vi "VIH Project - Get Effective Group Rule - Inherit.vi"(7 "Ignore Control Rules (F)":bool, 10 "Group Rule":T1, 11 "Parent Group Rule":T1) -> (2 "Effective Group Rule":T1)   [LabVIEW 2014]
doc: "::: VI Helpeks :::\nCopyright (c) 2000-2026 Konstantin Shifershteyn. All rights reserved."
uses:
  _VIH HelpGen.llb/VIH HelpGen Typedef - Cluster - Group Rule.ctl
  _VIH HelpGen.llb/VIH HelpGen Typedef - Enum - Default,Enable,Disable.ctl
  _VIH HelpGen.llb/VIH HelpGen Typedef - Cluster - Group Rule - Source Paths.ctl
  _VIH HelpGen.llb/VIH HelpGen Typedef - Cluster - Group Rule - Target Paths.ctl
  _VIH HelpGen.llb/VIH HelpGen Typedef - Enum - Description Mode.ctl
  _VIH HelpGen.llb/VIH HelpGen Typedef - Cluster - Control Rule.ctl
  _VIH HelpGen.llb/VIH HelpGen Typedef - Cluster - Enum Value Info.ctl
  _VIH HelpGen.llb/VIH HelpGen Typedef - Cluster - Group Rule - Flags.ctl
panel:
  # "VI Helpeks\nCopyright (c) 2012-2026 Konstantin Shifershteyn"
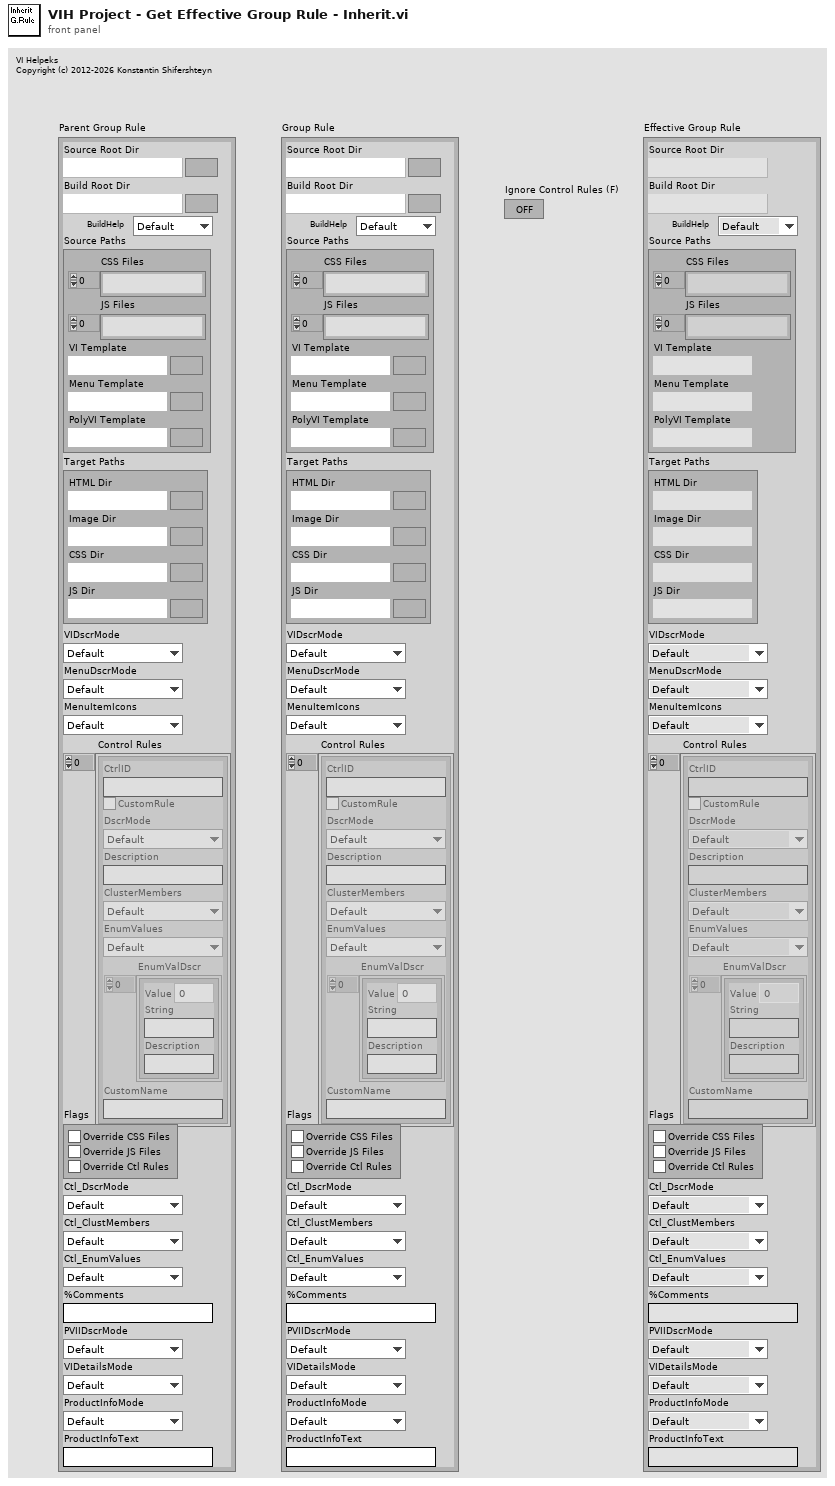
[diagram p1: front panel]
types:
  T1 = typedef "VIH HelpGen Typedef - Cluster - Group Rule.ctl" = cluster{"Source Root Dir":path, "Build Root Dir":path, "BuildHelp":T2, "Source Paths":T3, "Target Paths":T4, "VIDscrMode":T5, "MenuDscrMode":T5, "MenuItemIcons":T2, "Control Rules":T6[], "Flags":T8, "Ctl_DscrMode":T5, "Ctl_ClustMembers":T2, "Ctl_EnumValues":T2, "%Comments":string, "PVIIDscrMode":T5, "VIDetailsMode":T5, "ProductInfoMode":T2, "ProductInfoText":string}
  T2 = typedef "VIH HelpGen Typedef - Enum - Default,Enable,Disable.ctl" = enum16{"Default", "Enable", "Disable"}
  T3 = typedef "VIH HelpGen Typedef - Cluster - Group Rule - Source Paths.ctl" = cluster{"CSS Files":path[], "JS Files":path[], "VI Template":path, "Menu Template":path, "PolyVI Template":path}
  T4 = typedef "VIH HelpGen Typedef - Cluster - Group Rule - Target Paths.ctl" = cluster{"HTML Dir":path, "Image Dir":path, "CSS Dir":path, "JS Dir":path}
  T5 = typedef "VIH HelpGen Typedef - Enum - Description Mode.ctl" = enum16{"Default", "Description", "Description1", "Description2", "Custom", "None"}
  T6 = typedef "VIH HelpGen Typedef - Cluster - Control Rule.ctl" = cluster{"CtrlID":string, "CustomRule":bool, "DscrMode":T5, "Description":string, "ClusterMembers":T2, "EnumValues":T2, "EnumValDscr":T7[], "CustomName":string}
  T7 = typedef "VIH HelpGen Typedef - Cluster - Enum Value Info.ctl" = cluster{"Value":ext, "String":string, "Description":string}
  T8 = typedef "VIH HelpGen Typedef - Cluster - Group Rule - Flags.ctl" = cluster{"Override CSS Files":bool, "Override JS Files":bool, "Override Ctl Rules":bool}
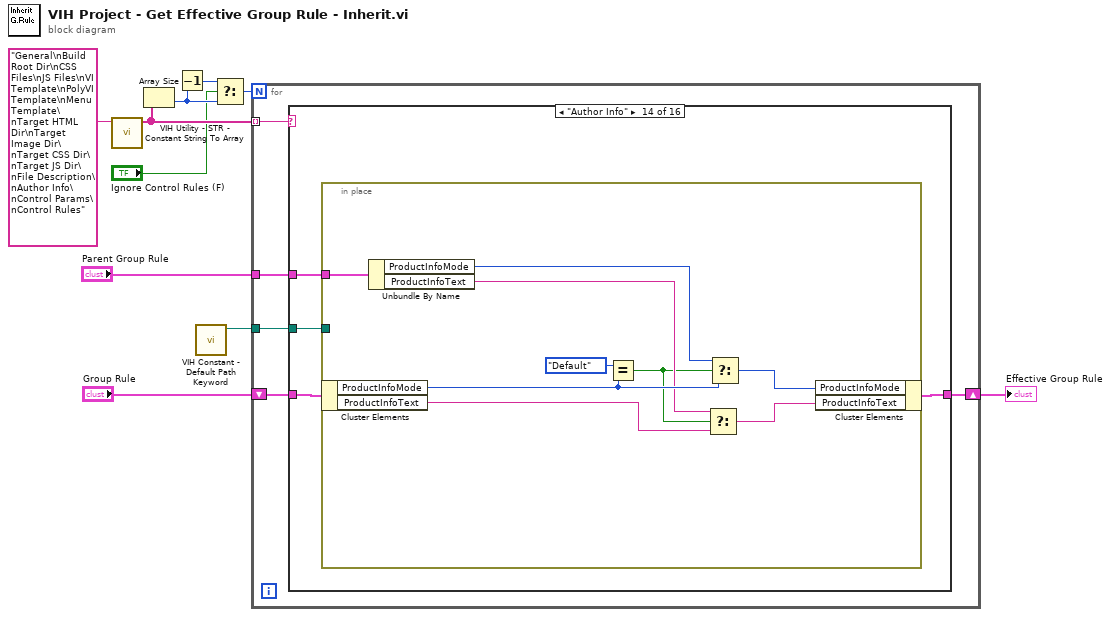
[diagram p0: block diagram]
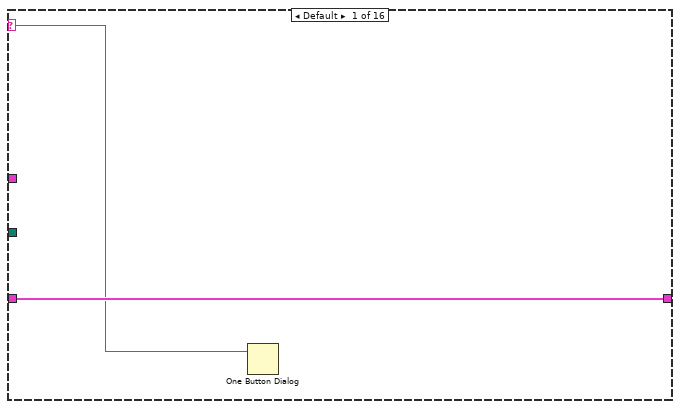
[diagram p2: hidden frame]
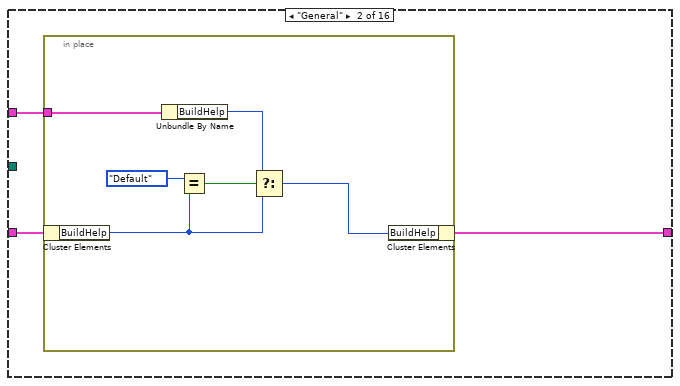
[diagram p3: hidden frame]
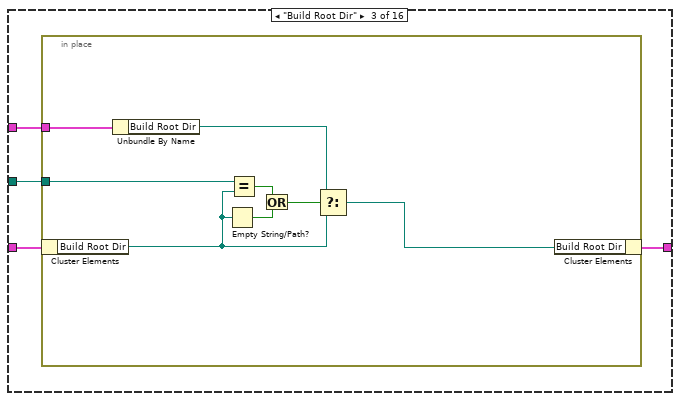
[diagram p4: hidden frame]
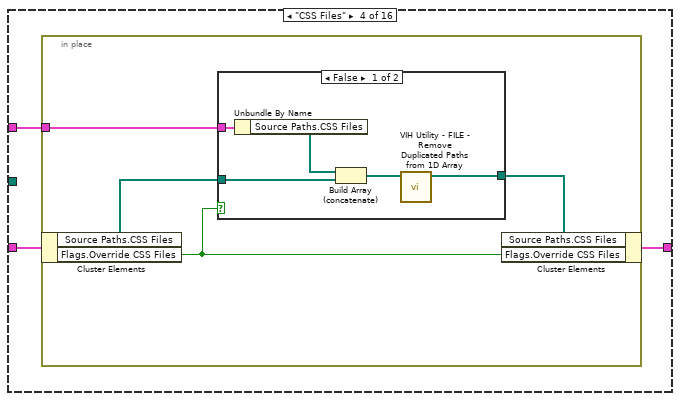
[diagram p5: hidden frame]
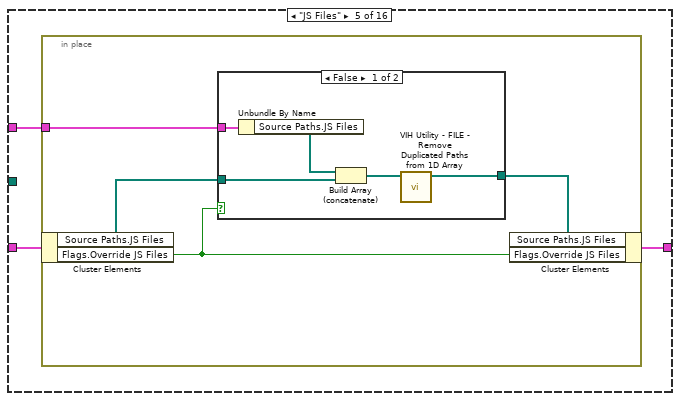
[diagram p7: hidden frame]
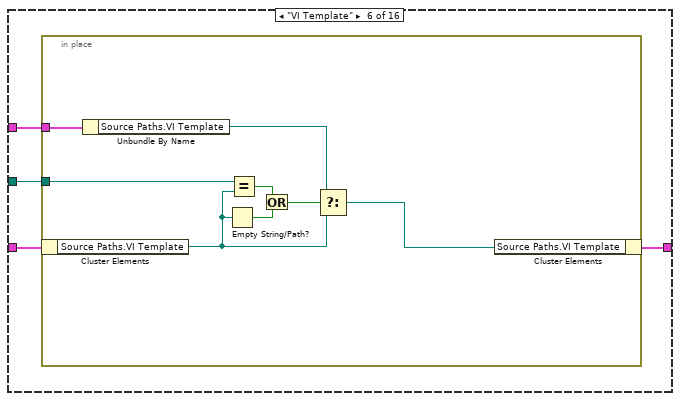
[diagram p9: hidden frame]
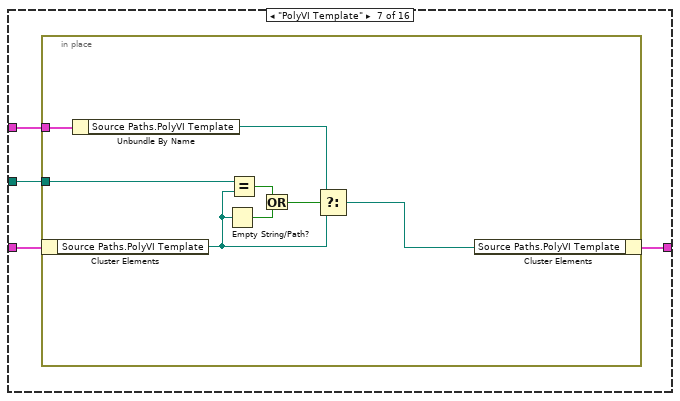
[diagram p10: hidden frame]
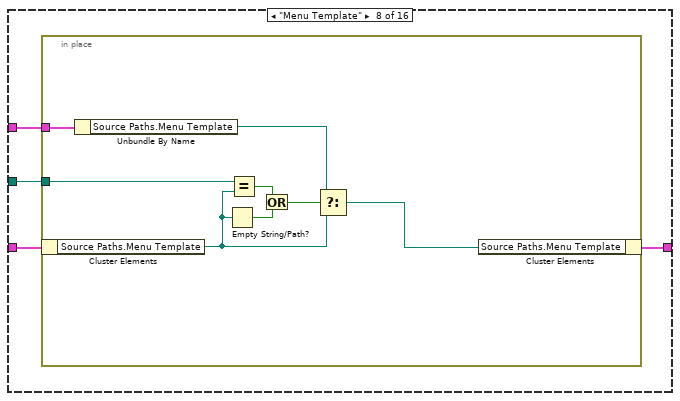
[diagram p11: hidden frame]
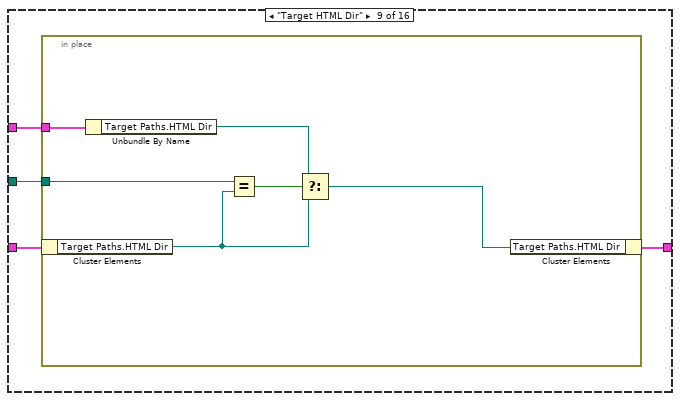
[diagram p12: hidden frame]
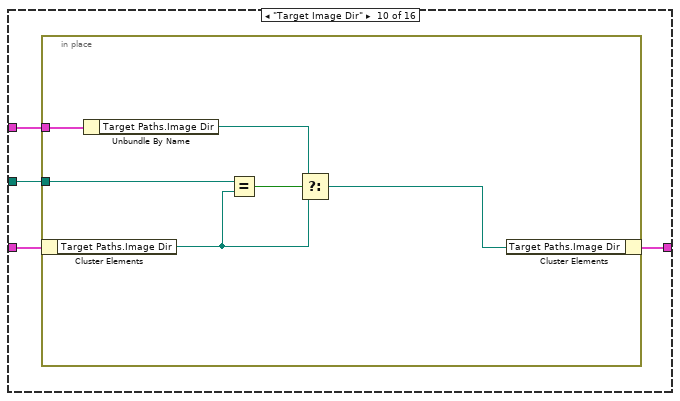
[diagram p13: hidden frame]
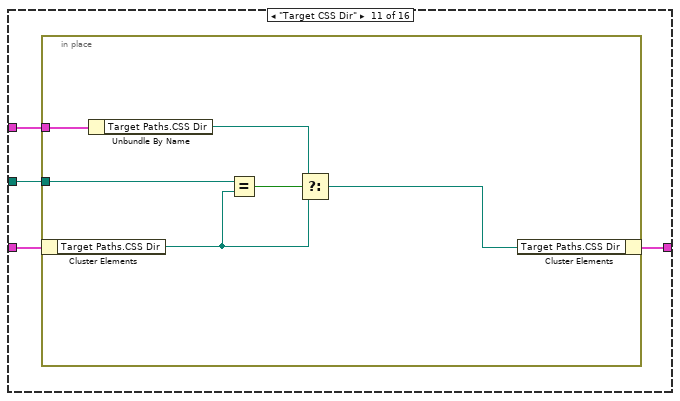
[diagram p14: hidden frame]
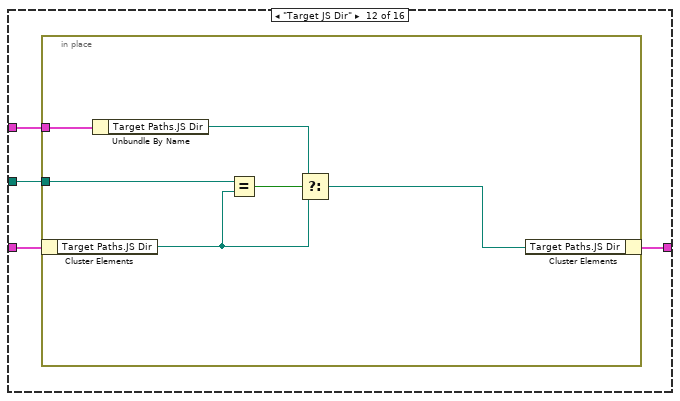
[diagram p15: hidden frame]
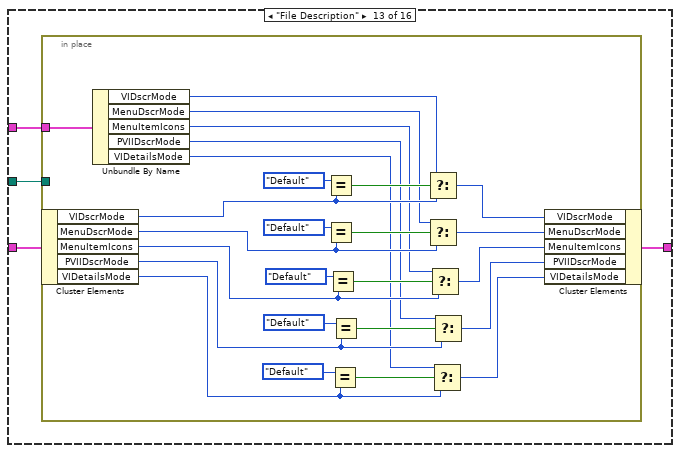
[diagram p16: hidden frame]
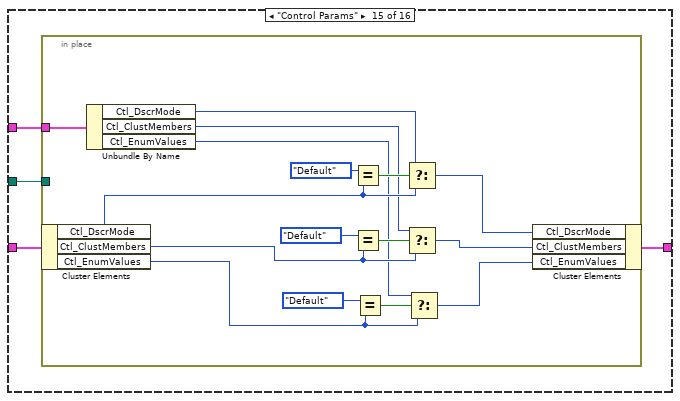
[diagram p17: hidden frame]
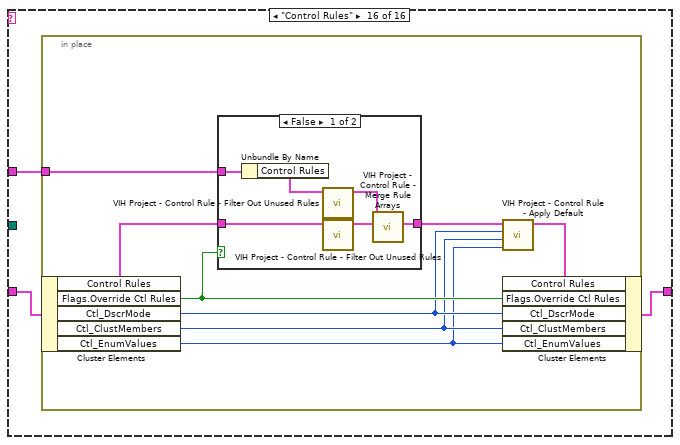
[diagram p18: hidden frame]
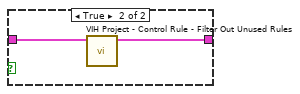
[diagram p19: hidden frame]
diagram:
  n1 = call "VIH Utility - STR - Constant String To Array.vi"("String in"="General\nBuild Root Dir\nCSS Files\nJS Files\nVI Template\nPolyVI Template\nMenu Template\nTarget HTML Dir\nTarget Image Dir\nTarget CSS Dir\nTarget JS Dir\nFile Description\nAuthor Info\nControl Params\nControl Rules") -> ("Array out"=w6:string[])  [unwired: 10 in]
  n2 = Array Size(array=w6) -> (size(s)=w4:i32)
  n3 = Decrement(x=w4) -> (x-1=w5:i32)
  n4 = call "VIH Constant - Default Path Keyword.vi"() -> ("<default> path"=w1:path)  [unwired: 11 in]
  n5 = Select(t=w5, s="Ignore Control Rules (F)", f=w4) -> (s? t:f=w2:i32)
  n6 = for {
    N: w2 -> [_]
    tunnel: w6 -> [w15] mode=indexing
    shift-right: [w14] -> w8
    shift-left: "Group Rule" -> [w13]
    tunnel: "Parent Group Rule" -> [w12]
    tunnel: w1 -> [w11]
    n7 = case shown="\"Author Info\"" w15 {
      selector: w15 -> [w16 _ _ _ _ _ _ _ _ _ _ _ _ _ _ _]
      tunnel: [w17 w19 w29 w40 w53 w67 w79 w91 w103 w113 w123 w133 w143 w173 w186 w205] -> w14
      tunnel: w13 -> [w17 w20 w30 w41 w54 w68 w80 w92 w104 w114 w124 w134 w144 w174 w187 w206]
      tunnel: w12 -> [_ w18 w28 w39 w52 w66 w78 w90 w102 w112 w122 w132 w142 w172 w185 w204]
      tunnel: w11 -> [_ _ w27 _ _ w65 w77 w89 w101 w111 w121 w131 w141 w171 w184 _]
      frame Default {
        n8 = One Button Dialog(message=w16) -> ()  [unwired: 1 in, 1 out]
      }
      frame "General" {
        n9 = in-place {
          in-place-border: w18 -> [w26]
          n10 = in-place-cluster #1(w20) -> ("BuildHelp"=w22:T2)
          n11 = Unbundle By Name(w26) -> ("BuildHelp"=w23:T2)
          n12 = Equal?(x=VIH_HelpGen_Typedef_-_Enum_-_Default,Enable,Disable."Default", y=w22) -> (x = y?=w24:bool)
          n13 = Select(t=w23, s=w24, f=w22) -> (s? t:f=w21:T2)
          n14 = in-place-cluster #1("BuildHelp"=w21) -> (w19:T1)
        }
      }
      frame "Build Root Dir" {
        n15 = in-place {
          in-place-border: w28 -> [w38]
          in-place-border: w27 -> [w31]
          n16 = in-place-cluster #2(w30) -> ("Build Root Dir"=w33:path)
          n17 = Unbundle By Name(w38) -> ("Build Root Dir"=w34:path)
          n18 = Empty String/Path?(string/path=w33) -> (empty?=w36:bool)
          n19 = Equal?(x=w31, y=w33) -> (x = y?=w37:bool)
          n20 = Or(x=w37, y=w36) -> (x .or. y?=w35:bool)
          n21 = Select(t=w34, s=w35, f=w33) -> (s? t:f=w32:path)
          n22 = in-place-cluster #2("Build Root Dir"=w32) -> (w29:T1)
        }
      }
      frame "CSS Files" {
        n23 = in-place {
          in-place-border: w39 -> [w45]
          n24 = in-place-cluster #3(w41) -> ("Source Paths.CSS Files"=w43:path[], "Flags.Override CSS Files"=w42:bool)
          n25 = case shown="False" w42 {
            tunnel: w45 -> [w50 _]
            tunnel: [w46 w51] -> w44
            tunnel: w43 -> [w49 w51]
            frame False {
              n26 = Unbundle By Name(w50) -> ("Source Paths.CSS Files"=w48:path[])
              n27 = Build Array (concatenate)(w48, w49) -> (w47:path[])
              n28 = call "VIH Utility - FILE - Remove Duplicated Paths from 1D Array.vi"("Array in"=w47) -> ("Array out"=w46:path[])  [unwired: 9 in, 1 out]
            }
            frame True {
            }
          }
          n29 = in-place-cluster #3("Source Paths.CSS Files"=w44, "Flags.Override CSS Files"=w42) -> (w40:T1)
        }
      }
      frame "JS Files" {
        n30 = in-place {
          in-place-border: w52 -> [w58]
          n31 = in-place-cluster #4(w54) -> ("Source Paths.JS Files"=w56:path[], "Flags.Override JS Files"=w55:bool)
          n32 = case shown="False" w55 {
            tunnel: w58 -> [w63 _]
            tunnel: [w59 w64] -> w57
            tunnel: w56 -> [w62 w64]
            frame False {
              n33 = Unbundle By Name(w63) -> ("Source Paths.JS Files"=w61:path[])
              n34 = Build Array (concatenate)(w61, w62) -> (w60:path[])
              n35 = call "VIH Utility - FILE - Remove Duplicated Paths from 1D Array.vi"("Array in"=w60) -> ("Array out"=w59:path[])  [unwired: 9 in, 1 out]
            }
            frame True {
            }
          }
          n36 = in-place-cluster #4("Source Paths.JS Files"=w57, "Flags.Override JS Files"=w55) -> (w53:T1)
        }
      }
      frame "VI Template" {
        n37 = in-place {
          in-place-border: w66 -> [w76]
          in-place-border: w65 -> [w69]
          n38 = in-place-cluster #5(w68) -> ("Source Paths.VI Template"=w71:path)
          n39 = Unbundle By Name(w76) -> ("Source Paths.VI Template"=w72:path)
          n40 = Empty String/Path?(string/path=w71) -> (empty?=w74:bool)
          n41 = Equal?(x=w69, y=w71) -> (x = y?=w75:bool)
          n42 = Or(x=w75, y=w74) -> (x .or. y?=w73:bool)
          n43 = Select(t=w72, s=w73, f=w71) -> (s? t:f=w70:path)
          n44 = in-place-cluster #5("Source Paths.VI Template"=w70) -> (w67:T1)
        }
      }
      frame "PolyVI Template" {
        n45 = in-place {
          in-place-border: w78 -> [w88]
          in-place-border: w77 -> [w81]
          n46 = in-place-cluster #6(w80) -> ("Source Paths.PolyVI Template"=w83:path)
          n47 = Unbundle By Name(w88) -> ("Source Paths.PolyVI Template"=w84:path)
          n48 = Empty String/Path?(string/path=w83) -> (empty?=w86:bool)
          n49 = Equal?(x=w81, y=w83) -> (x = y?=w87:bool)
          n50 = Or(x=w87, y=w86) -> (x .or. y?=w85:bool)
          n51 = Select(t=w84, s=w85, f=w83) -> (s? t:f=w82:path)
          n52 = in-place-cluster #6("Source Paths.PolyVI Template"=w82) -> (w79:T1)
        }
      }
      frame "Menu Template" {
        n53 = in-place {
          in-place-border: w90 -> [w100]
          in-place-border: w89 -> [w93]
          n54 = in-place-cluster #7(w92) -> ("Source Paths.Menu Template"=w95:path)
          n55 = Unbundle By Name(w100) -> ("Source Paths.Menu Template"=w96:path)
          n56 = Empty String/Path?(string/path=w95) -> (empty?=w98:bool)
          n57 = Equal?(x=w93, y=w95) -> (x = y?=w99:bool)
          n58 = Or(x=w99, y=w98) -> (x .or. y?=w97:bool)
          n59 = Select(t=w96, s=w97, f=w95) -> (s? t:f=w94:path)
          n60 = in-place-cluster #7("Source Paths.Menu Template"=w94) -> (w91:T1)
        }
      }
      frame "Target HTML Dir" {
        n61 = in-place {
          in-place-border: w102 -> [w110]
          in-place-border: w101 -> [w106]
          n62 = in-place-cluster #8(w104) -> ("Target Paths.HTML Dir"=w108:path)
          n63 = Unbundle By Name(w110) -> ("Target Paths.HTML Dir"=w109:path)
          n64 = Equal?(x=w106, y=w108) -> (x = y?=w105:bool)
          n65 = Select(t=w109, s=w105, f=w108) -> (s? t:f=w107:path)
          n66 = in-place-cluster #8("Target Paths.HTML Dir"=w107) -> (w103:T1)
        }
      }
      frame "Target Image Dir" {
        n67 = in-place {
          in-place-border: w112 -> [w120]
          in-place-border: w111 -> [w116]
          n68 = in-place-cluster #9(w114) -> ("Target Paths.Image Dir"=w118:path)
          n69 = Unbundle By Name(w120) -> ("Target Paths.Image Dir"=w119:path)
          n70 = Equal?(x=w116, y=w118) -> (x = y?=w115:bool)
          n71 = Select(t=w119, s=w115, f=w118) -> (s? t:f=w117:path)
          n72 = in-place-cluster #9("Target Paths.Image Dir"=w117) -> (w113:T1)
        }
      }
      frame "Target CSS Dir" {
        n73 = in-place {
          in-place-border: w122 -> [w130]
          in-place-border: w121 -> [w126]
          n74 = in-place-cluster #10(w124) -> ("Target Paths.CSS Dir"=w128:path)
          n75 = Unbundle By Name(w130) -> ("Target Paths.CSS Dir"=w129:path)
          n76 = Equal?(x=w126, y=w128) -> (x = y?=w125:bool)
          n77 = Select(t=w129, s=w125, f=w128) -> (s? t:f=w127:path)
          n78 = in-place-cluster #10("Target Paths.CSS Dir"=w127) -> (w123:T1)
        }
      }
      frame "Target JS Dir" {
        n79 = in-place {
          in-place-border: w132 -> [w140]
          in-place-border: w131 -> [w136]
          n80 = in-place-cluster #11(w134) -> ("Target Paths.JS Dir"=w138:path)
          n81 = Unbundle By Name(w140) -> ("Target Paths.JS Dir"=w139:path)
          n82 = Equal?(x=w136, y=w138) -> (x = y?=w135:bool)
          n83 = Select(t=w139, s=w135, f=w138) -> (s? t:f=w137:path)
          n84 = in-place-cluster #11("Target Paths.JS Dir"=w137) -> (w133:T1)
        }
      }
      frame "File Description" {
        n85 = in-place {
          in-place-border: w142 -> [w170]
          in-place-border: w141 -> [_]
          n86 = in-place-cluster #12(w144) -> ("VIDscrMode"=w168:T5, "MenuDscrMode"=w161:T5, "MenuItemIcons"=w160:T2, "PVIIDscrMode"=w153:T5, "VIDetailsMode"=w147:T5)
          n87 = Unbundle By Name(w170) -> ("VIDscrMode"=w169:T5, "MenuDscrMode"=w158:T5, "MenuItemIcons"=w157:T2, "PVIIDscrMode"=w152:T5, "VIDetailsMode"=w146:T5)
          n88 = Equal?(x=VIH_HelpGen_Typedef_-_Enum_-_Description_Mode."Default", y=w168) -> (x = y?=w166:bool)
          n89 = Equal?(x=VIH_HelpGen_Typedef_-_Enum_-_Description_Mode."Default", y=w161) -> (x = y?=w163:bool)
          n90 = Equal?(x=VIH_HelpGen_Typedef_-_Enum_-_Default,Enable,Disable."Default", y=w160) -> (x = y?=w162:bool)
          n91 = Equal?(x=VIH_HelpGen_Typedef_-_Enum_-_Description_Mode."Default", y=w147) -> (x = y?=w148:bool)
          n92 = Equal?(x=VIH_HelpGen_Typedef_-_Enum_-_Description_Mode."Default", y=w153) -> (x = y?=w154:bool)
          n93 = Select(t=w169, s=w166, f=w168) -> (s? t:f=w167:T5)
          n94 = Select(t=w158, s=w163, f=w161) -> (s? t:f=w156:T5)
          n95 = Select(t=w157, s=w162, f=w160) -> (s? t:f=w155:T2)
          n96 = Select(t=w146, s=w148, f=w147) -> (s? t:f=w145:T5)
          n97 = Select(t=w152, s=w154, f=w153) -> (s? t:f=w151:T5)
          n98 = in-place-cluster #12("VIDscrMode"=w167, "MenuDscrMode"=w156, "MenuItemIcons"=w155, "PVIIDscrMode"=w151, "VIDetailsMode"=w145) -> (w143:T1)
        }
      }
      frame "Author Info" {
        n99 = in-place {
          in-place-border: w172 -> [w183]
          in-place-border: w171 -> [_]
          n100 = in-place-cluster #13(w174) -> ("ProductInfoMode"=w182:T2, "ProductInfoText"=w176:string)
          n101 = Unbundle By Name(w183) -> ("ProductInfoMode"=w180:T2, "ProductInfoText"=w178:string)
          n102 = Equal?(x=VIH_HelpGen_Typedef_-_Enum_-_Default,Enable,Disable."Default", y=w182) -> (x = y?=w177:bool)
          n103 = Select(t=w178, s=w177, f=w176) -> (s? t:f=w175:string)
          n104 = Select(t=w180, s=w177, f=w182) -> (s? t:f=w179:T2)
          n105 = in-place-cluster #13("ProductInfoMode"=w179, "ProductInfoText"=w175) -> (w173:T1)
        }
      }
      frame "Control Params" {
        n106 = in-place {
          in-place-border: w185 -> [w203]
          in-place-border: w184 -> [_]
          n107 = in-place-cluster #14(w187) -> ("Ctl_DscrMode"=w201:T5, "Ctl_ClustMembers"=w195:T2, "Ctl_EnumValues"=w194:T2)
          n108 = Unbundle By Name(w203) -> ("Ctl_DscrMode"=w202:T5, "Ctl_ClustMembers"=w192:T2, "Ctl_EnumValues"=w191:T2)
          n109 = Equal?(x=VIH_HelpGen_Typedef_-_Enum_-_Description_Mode."Default", y=w201) -> (x = y?=w199:bool)
          n110 = Equal?(x=VIH_HelpGen_Typedef_-_Enum_-_Default,Enable,Disable."Default", y=w195) -> (x = y?=w197:bool)
          n111 = Equal?(x=VIH_HelpGen_Typedef_-_Enum_-_Default,Enable,Disable."Default", y=w194) -> (x = y?=w196:bool)
          n112 = Select(t=w202, s=w199, f=w201) -> (s? t:f=w200:T5)
          n113 = Select(t=w192, s=w197, f=w195) -> (s? t:f=w190:T2)
          n114 = Select(t=w191, s=w196, f=w194) -> (s? t:f=w189:T2)
          n115 = in-place-cluster #14("Ctl_DscrMode"=w200, "Ctl_ClustMembers"=w190, "Ctl_EnumValues"=w189) -> (w186:T1)
        }
      }
      frame "Control Rules" {
        n116 = in-place {
          in-place-border: w204 -> [w214]
          n117 = in-place-cluster #15(w206) -> ("Control Rules"=w213:T6[], "Flags.Override Ctl Rules"=w212:bool, "Ctl_DscrMode"=w209:T5, "Ctl_ClustMembers"=w208:T2, "Ctl_EnumValues"=w207:T2)
          n118 = case shown="False" w212 {
            tunnel: w214 -> [w220 _]
            tunnel: [w215 w221] -> w211
            tunnel: w213 -> [w218 w222]
            frame False {
              n119 = Unbundle By Name(w220) -> ("Control Rules"=w219:T6[])
              n120 = call "VIH Project - Control Rule - Filter Out Unused Rules.vi"("Control Rules"=w219) -> ("Control Rules out"=w216:T6[])  [unwired: 10 in]
              n121 = call "VIH Project - Control Rule - Filter Out Unused Rules.vi"("Control Rules"=w218) -> ("Control Rules out"=w217:T6[])  [unwired: 10 in]
              n122 = call "VIH Project - Control Rule - Merge Rule Arrays.vi"("Control Rules"=w217, "Parent Control Rules"=w216) -> ("Control Rules out"=w215:T6[])  [unwired: 9 in]
            }
            frame True {
              n123 = call "VIH Project - Control Rule - Filter Out Unused Rules.vi"("Control Rules"=w222) -> ("Control Rules out"=w221:T6[])  [unwired: 10 in]
            }
          }
          n124 = call "VIH Project - Control Rule - Apply Default.vi"("default EnumValues"=w207, "default ClusterMembers"=w208, "default DscrMode"=w209, "Control Rules"=w211) -> ("Control Rules out"=w210:T6[])  [unwired: 7 in]
          n125 = in-place-cluster #15("Control Rules"=w210, "Flags.Override Ctl Rules"=w212, "Ctl_DscrMode"=w209, "Ctl_ClustMembers"=w208, "Ctl_EnumValues"=w207) -> (w205:T1)
        }
      }
    }
  }
  "Effective Group Rule" <- w8
